vi "Create LVClass for Oneof.vi"(7 "Message Elements":T1[](array[typedef]), 8 "error in (no error)":errorcluster, 9 "Message Name":string, 10 "Parent Message Typedef":refnum<vi>, 11 "Library":refnum<vi>) -> (0 "error out":errorcluster, 3 "Library":refnum<vi>)   [LabVIEW 2019, in "gRPC Template Creation Utility.lvlib"]
uses:
  gRPC Template Creation Utility.lvlib
  TypeDefs/Message Element Metadata (Scripting).ctl
  TypeDefs/Message Element Type.ctl
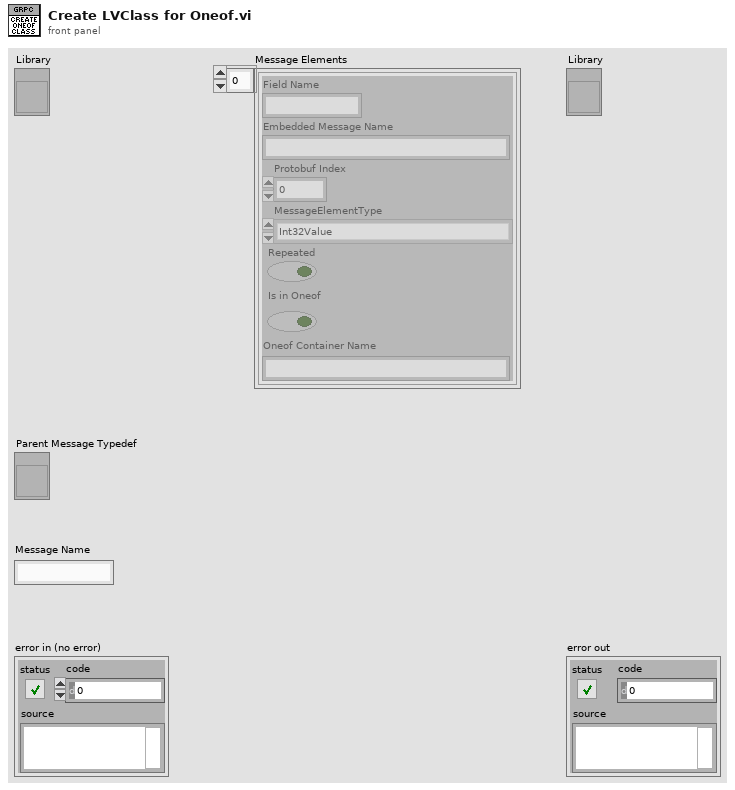
[diagram p1: front panel]
types:
  T1 = typedef "gRPC Template Creation Utility.lvlib/Message Element Metadata (Scripting).ctl" = cluster{"Field Name":string, "Embedded Message Name":string, "Protobuf Index":i32, "MessageElementType":T2, "Repeated":bool, "Is in Oneof":bool, "Oneof Container Name":string}
  T2 = typedef "gRPC Template Creation Utility.lvlib/Message Element Type.ctl" = enum32{"Int32Value", "FloatValue", "DoubleValue", "BoolValue", "StringValue", "MessageValue", "Int64Value", "UInt32Value", "UInt64Value", "EnumValue", "Bytes", "Fixed64", "Fixed32", "SFixed64", "SFixed32", "SInt64", "SInt32"}
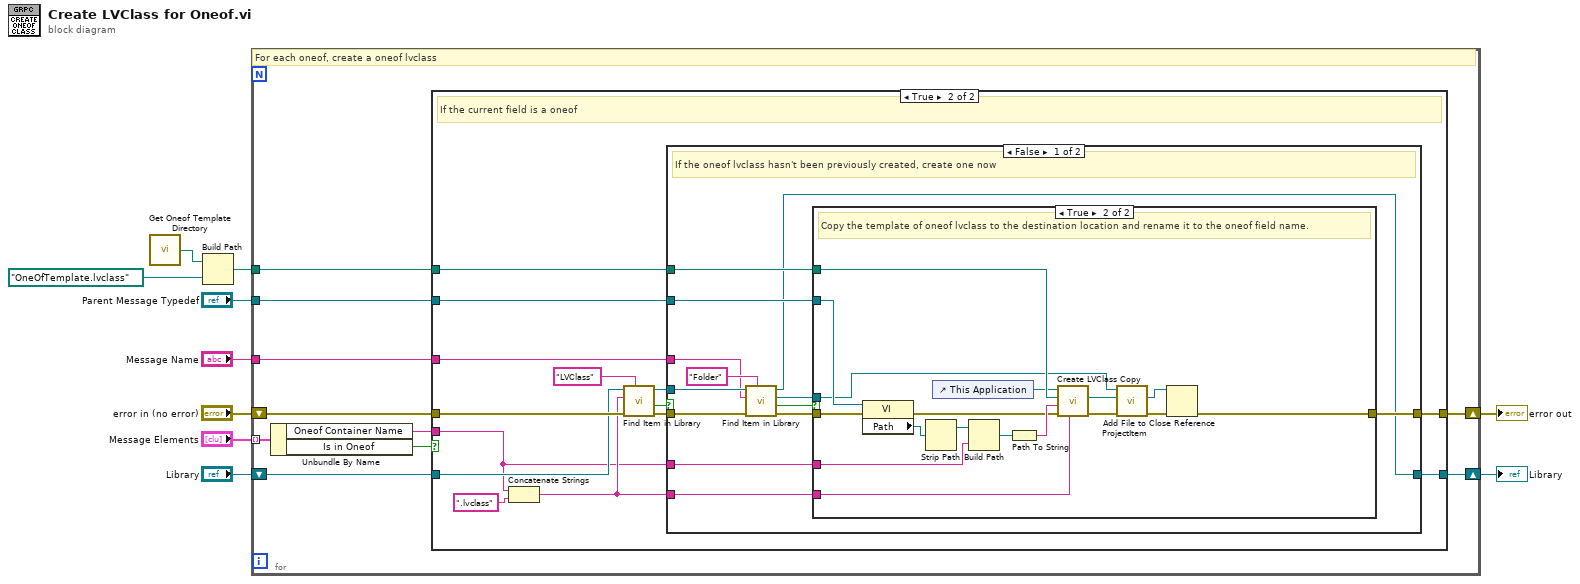
[diagram p0: block diagram]
diagram:
  n1 = call "Get Oneof Template Directory.vi"() -> ("appended path"=w3:path)
  n2 = Build Path(base path=w3, name or relative path=path "OneOfTemplate.lvclass") -> (appended path=w2:path)
  n3 = for {
    tunnel: "Message Elements" -> [w20] mode=indexing
    tunnel: "Message Name" -> [w16]
    tunnel: "Parent Message Typedef" -> [w13]
    tunnel: w2 -> [w12]
    shift-right: [w17] -> w9
    shift-left: "error in (no error)" -> [w18]
    shift-right: [w14] -> w6
    shift-left: "Library" -> [w15]
    # "For each oneof, create a oneof lvclass"
    n4 = Unbundle By Name(w20) -> ("Oneof Container Name"=w11:string, "Is in Oneof"=w19:bool)
    n5 = case shown="True" w19 {
      tunnel: [w22 w36] -> w17
      tunnel: w18 -> [w22 w33]
      tunnel: w16 -> [_ w35]
      tunnel: w15 -> [w21 w32]
      tunnel: [w21 w34] -> w14
      tunnel: w13 -> [_ w26]
      tunnel: w12 -> [_ w25]
      tunnel: w11 -> [_ w23]
      frame False {
      }
      frame True {
        # "If the current field is a oneof"
        n6 = Concatenate Strings(w23, ".lvclass" ("string")) -> (w24:string)
        n7 = call "Find Item in Library.vi"("Item Type"="LVClass", "error in (no error)"=w33, "Item Name"=w24, "Library item in"=w32) -> ("error out"=w28:errorcluster, "Found?"=w27:bool, "Library item out"=w31:refnum<vi>)  [unwired: 4 in, 1 out]
        n8 = case shown="False" w27 {
          tunnel: [w45 w68] -> w36
          tunnel: w23 -> [w44 _]
          tunnel: w35 -> [w41 _]
          tunnel: [w37 w69] -> w34
          tunnel: w31 -> [w42 w69]
          tunnel: w28 -> [w43 w68]
          tunnel: w26 -> [w40 _]
          tunnel: w25 -> [w39 _]
          tunnel: w24 -> [w38 _]
          frame False {
            # "If the oneof lvclass hasn't been previously created, create one now"
            n9 = call "Find Item in Library.vi"("Item Type"="Folder", "error in (no error)"=w43, "Item Name"=w41, "Library item in"=w42) -> ("error out"=w47:errorcluster, "Found?"=w46:bool, "Project Item (Library Item)"=w49:refnum<vi>, "Library item out"=w37:refnum<vi>)  [unwired: 4 in]
            n10 = case shown="True" w46 {
              tunnel: w44 -> [_ w54]
              tunnel: w49 -> [_ w51]
              tunnel: [w50 w64] -> w45
              tunnel: w47 -> [w50 w60]
              tunnel: w40 -> [_ w65]
              tunnel: w39 -> [_ w62]
              tunnel: w38 -> [_ w53]
              frame False {
                # "Container message should have been created already."
              }
              frame True {
                # "Copy the template of oneof lvclass to the destination location and rename it to the oneof field name."
                n11 = property class="VI"(reference=w65, error in=w60) -> (error out=w59:errorcluster, "Path"=w66:path)  [unwired: 1 out]
                n12 = Strip Path(path=w66) -> (stripped path=w56:path)  [unwired: 1 out]
                n13 = control-ref of="This Application"() -> (w57:refnum<vi>)
                n14 = Build Path(base path=w56, name or relative path=w54) -> (appended path=w55:path)
                n15 = Path To String(path=w55) -> (string=w61:string)
                n16 = call "Create LVClass Copy.vi"("New Name"=w53, "error in (no error)"=w59, "New Path"=w61, "Source Class Path"=w62, "Application in"=w57) -> ("error out"=w58:errorcluster, "Copy Class Path out"=w52:path)  [unwired: 4 in, 1 out]
                n17 = call "Add File to ProjectItem.vi"("error in (no error)"=w58, "File Path"=w52, "ProjectItem in"=w51) -> ("error out"=w63:errorcluster, "Added File ref"=w67:refnum<vi>)  [unwired: 6 in, 1 out]
                n18 = Close Reference(reference=w67, error in (no error)=w63) -> (error out=w64:errorcluster)
              }
            }
          }
          frame True {
          }
        }
      }
    }
  }
  "error out" <- w9
  "Library" <- w6
